vi "Create Toast Notifier.vi"(8 "error in":errorcluster) -> (0 "error out":errorcluster, 3 "Toast Notifier":refnum<k24>)   [LabVIEW 2026, in "ToastNotification.lvlib" / "Toast Native.lvlib"]
doc: "Find Microsoft.Toolkit.Uwp.Notifications.dll under the toolkit root, resolve ToastNotificationManagerCompat from that assembly file and invoke CreateToastNotifier. Skips work on incoming error. The caller owns the returned Toast Notifier. Temporary reflection references are released after use."
uses:
  Toast Native.lvlib
  <vilib>/Utility/error.llb/Error Cluster From Error Code.vi
  <vilib>/ErrorRing/Error Ring.xnode
  Reflection DotNet/Reflection DotNet.lvlib
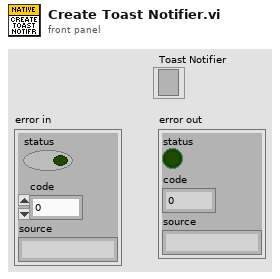
[diagram p1: front panel]
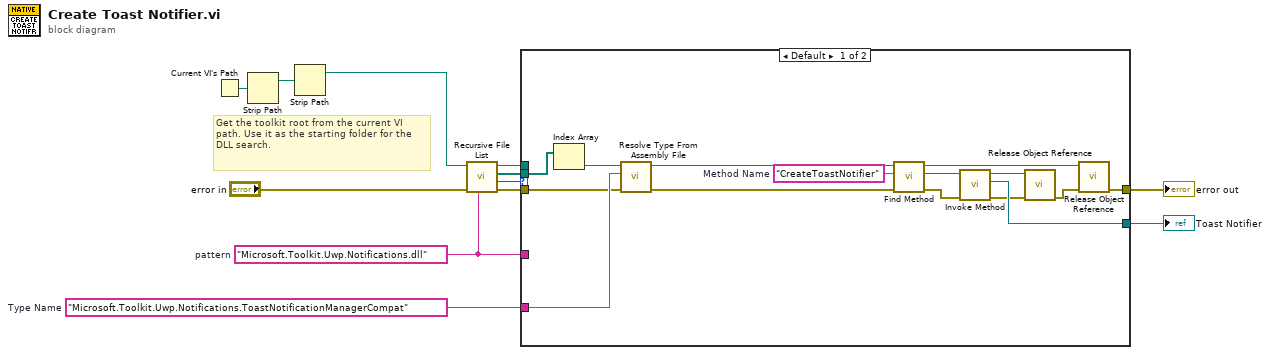
[diagram p0: block diagram]
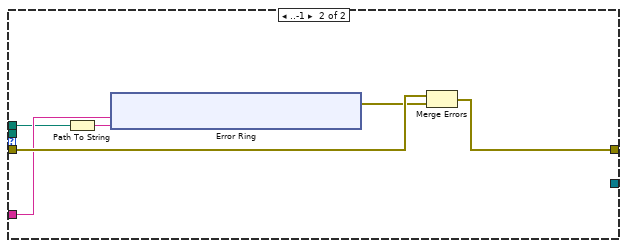
[diagram p2: hidden frame]
diagram:
  w4 = "Microsoft.Toolkit.Uwp.Notifications.dll"  # pattern
  w10 = "Microsoft.Toolkit.Uwp.Notifications.ToastNotificationManagerCompat"  # Type Name
  # "Get the toolkit root from the current VI path. Use it as the starting folder for the DLL search."
  n1 = Current VI's Path() -> (path=w3:path)
  n2 = Strip Path(path=w3) -> (stripped path=w2:path)  [unwired: 1 out]
  n3 = Strip Path(path=w2) -> (stripped path=w1:path)  [unwired: 1 out]
  n4 = call <vilib>:"Recursive File List.vi"("pattern"=w4, "error in (no error)"="error in", "Folder Path"=w1) -> ("error out"=w8:errorcluster, "Number of Files"=w7:i32, "All Files in Dir"=w6:path[], "dup Folder Path"=w5:path)  [unwired: 4 in, 1 out]
  n5 = case shown="Default" w7 {
    tunnel: [w24 _] -> w12
    tunnel: [w19 w33] -> w11
    tunnel: w10 -> [w17 _]
    tunnel: w8 -> [w15 w32]
    tunnel: w6 -> [w14 _]
    tunnel: w5 -> [_ w29]
    tunnel: w4 -> [_ w30]
    frame Default {
      w27 = "CreateToastNotifier"  # Method Name
      n6 = Index Array(array=w14) -> (element=w13:path)  [unwired: 1 in]
      n7 = call "Resolve Type From Assembly File.vi"("error in (no error)"=w15, "Type Name"=w17, "AssemblyFile"=w13) -> ("error out"=w18:errorcluster, "GetType out"=w16:refnum<k24>)  [unwired: 7 in]
      n8 = call "Find Method.vi"("error in (no error)"=w18, "Method Name"=w27, "Declaring Type in"=w16) -> ("error out"=w26:errorcluster, "Method Info"=w25:refnum<k24>, "Declaring Type out"=w21:refnum<k24>)  [unwired: 6 in]
      n9 = call "Invoke Method.vi"("error in (no error)"=w26, "Method Info in"=w25) -> ("error out"=w23:errorcluster, "Return Value"=w24:refnum<k24>, "Method Info out"=w22:refnum<k24>)  [unwired: 7 in]
      n10 = call "Release Object Reference.vi"("error in"=w23, "object"=w22) -> ("error out"=w20:errorcluster)  [unwired: 9 in]
      n11 = call "Release Object Reference.vi"("error in"=w20, "object"=w21) -> ("error out"=w19:errorcluster)  [unwired: 9 in]
    }
    frame ..-1 {
      n12 = Path To String(path=w29) -> (string=w28:string)
      n13 = xnode "Error Ring"("parameter 0"=w30, "parameter 1"=w28) -> ("error out"=w31:errorcluster)
      n14 = Merge Errors(w32, w31) -> (w33:errorcluster)
    }
  }
  "Toast Notifier" <- w12
  "error out" <- w11
